vi "VM Spy - build variable list shortcut menu.vi"(6 "Variable List mode (T)":bool=TRUE, 9 "Coords":T1, 10 "MenuRef":refnum<k9>, 11 "CtlRef":refnum<vi>) -> (0 "Discard menu":bool)   [LabVIEW 2021]
doc: "::: CalcExpress Toolkit :::\nCopyright (c) 2000-2026 Konstantin Shifershteyn. All rights reserved."
uses:
  <vilib>/Utility/miscctls.llb/LVPoint32TypeDef.ctl
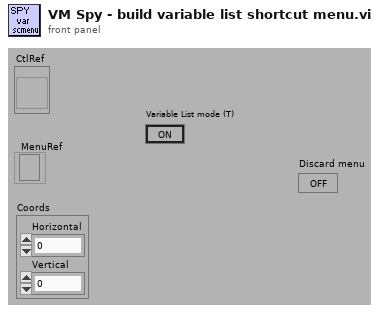
[diagram p1: front panel]
types:
  T1 = typedef "LVPoint32TypeDef.ctl" = cluster{"Horizontal":i32, "Vertical":i32}
  T2 = typedef "LVRowAndColumnTypeDef.ctl" = cluster{"Row":i32, "Column":i32}
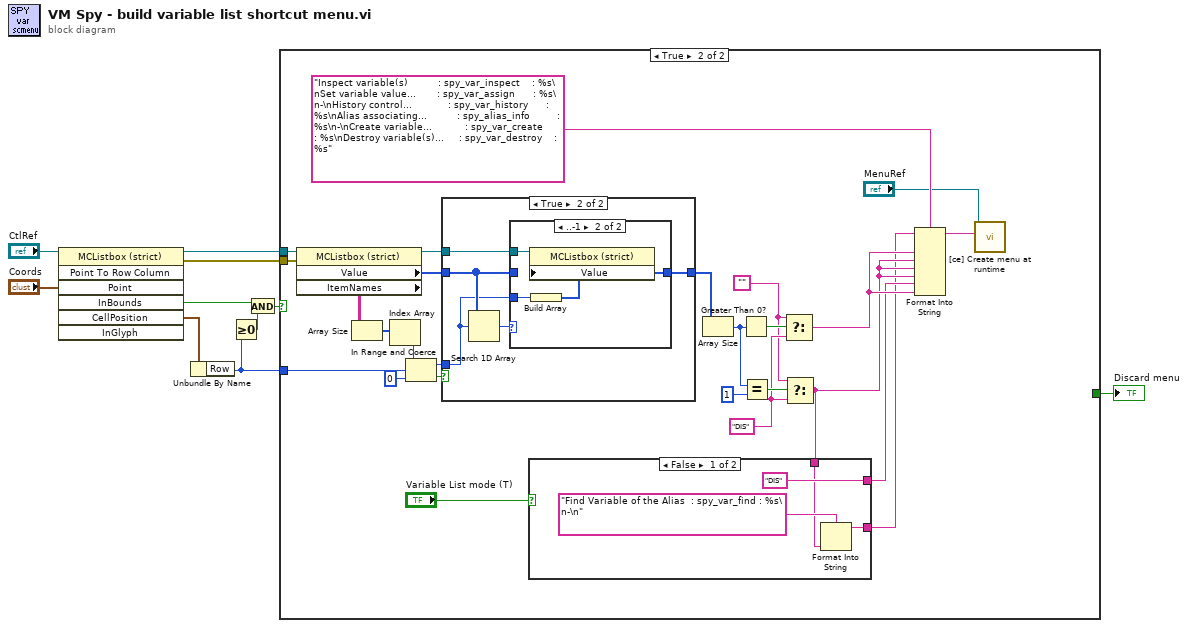
[diagram p0: block diagram]
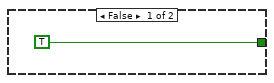
[diagram p2: hidden frame]
diagram:
  n1 = invoke class="MCListbox (strict)" method="Point To Row Column"(reference="CtlRef", "Point"="Coords") -> (reference out=w8:refnum<vi>, error out=w7:errorcluster, "InBounds"=w5:bool, "CellPosition"=w2:T2)  [unwired: 5 in, 3 out]
  n2 = Unbundle By Name(w2) -> ("Row"=w1:i32)
  n3 = Greater Or Equal To 0?(x=w1) -> (x >= 0?=w3:bool)
  n4 = And(x=w5, y=w3) -> (x .and. y?=w4:bool)
  n5 = case shown="True" w4 {
    tunnel: w8 -> [_ w37]
    tunnel: w7 -> [_ w36]
    tunnel: [TRUE _] -> w6
    tunnel: w1 -> [_ w23]
    frame False {
    }
    frame True {
      w19 = "DIS"
      w18 = ""
      n6 = property class="MCListbox (strict)"(reference=w37, error in=w36) -> (reference out=w28:refnum<vi>, "Value"=w29:i32[], "ItemNames"=w34:string[][])  [unwired: 1 out]
      n7 = Array Size(array=w34) -> (size(s)=w35:i32[])
      n8 = Index Array(array=w35) -> (element=w33:i32)  [unwired: 1 in]
      n9 = In Range and Coerce(upper limit=w33, x=w23, lower limit=0) -> (coerced(x)=w30:i32, In Range?=w31:bool)
      n10 = case shown="True" w31 {
        tunnel: w30 -> [_ w43]
        tunnel: w29 -> [_ w44]
        tunnel: w28 -> [_ w46]
        tunnel: [_ w42] -> w27
        frame False {
        }
        frame True {
          n11 = Search 1D Array(1D array=w44, element=w43) -> (index of element=w45:i32)  [unwired: 1 in]
          n12 = case shown="..-1" w45 {
            tunnel: w46 -> [_ w50]
            tunnel: [w47 w48] -> w42
            tunnel: w44 -> [w47 _]
            tunnel: w43 -> [_ w49]
            frame 0.. {
            }
            frame ..-1 {
              n13 = Build Array(w49) -> (w48:i32[])
              n14 = property class="MCListbox (strict)"(reference=w50, "Value"=w48) -> ()  [unwired: 1 in, 2 out]
            }
          }
        }
      }
      n15 = Array Size(array=w27) -> (size(s)=w21:i32)
      n16 = Greater Than 0?(x=w21) -> (x > 0?=w25:bool)
      n17 = Equal?(x=w21, y=1) -> (x = y?=w22:bool)
      n18 = Select(t=w18, s=w25, f=w19) -> (s? t:f=w17:string)
      n19 = Select(t=w18, s=w22, f=w19) -> (s? t:f=w14:string)
      n20 = case shown="False" "Variable List mode (T)" {
        tunnel: ["DIS" _] -> w15
        tunnel: [w39 _] -> w12
        tunnel: w14 -> [w38 _]
        frame False {
          n21 = Format Into String(format string="Find Variable of the Alias  : spy_var_find : %s\n-\n", w38) -> (resulting string=w39:string)  [unwired: 2 in, 1 out]
        }
        frame True {
        }
      }
      n22 = Format Into String(format string="Inspect variable(s)          : spy_var_inspect    : %s\nSet variable value...       : spy_var_assign      : %s\n-\nHistory control...            : spy_var_history      : %s\nAlias associating...          : spy_alias_info         : %s\n-\nCreate variable...           : spy_var_create      : %s\nDestroy variable(s)...     : spy_var_destroy    : %s", initial string=w12, w17, w14, w14, w14, w15, w17) -> (resulting string=w13:string)  [unwired: 1 in, 1 out]
      n23 = call "[ce] Create menu at runtime.vi"("menu descriptor"=w13, "menu"="MenuRef") -> ()  [unwired: 8 in, 2 out]
    }
  }
  "Discard menu" <- w6
